vi "Make PUT Object Request Parameters.vi"(11 "PUT Object Request Parameters":T1={"Content Type"="binary/octet-stream", "ACL"=enum."private", "Storage Class"=enum."STANDARD", "User-Defined Metadata"=[]}) -> (3 "HTTP Headers":T4[](array[typedef]))   [LabVIEW 2015, in "NI_AWS_S3.lvlib" / "Object.lvlib"]
uses:
  Object.lvlib
  Core/HTTP Request/Name Value Pair.ctl
  PUT Object Request Parameters.ctl
  ACL.ctl
  Storage Class.ctl
  Core/HTTP Request/HTTP Request.lvclass
  NI_AWS_S3.lvlib
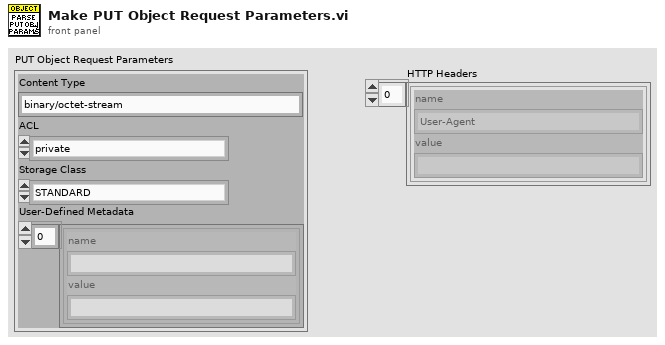
[diagram p1: front panel]
types:
  T1 = typedef "NI_AWS_S3.lvlib/PUT Object Request Parameters.ctl" = cluster{"Content Type":string, "ACL":T2, "Storage Class":T3, "User-Defined Metadata":T4[]}
  T2 = typedef "NI_AWS_S3.lvlib/ACL.ctl" = enum16{"private", "public-read", "public-read-write", "aws-exec-read", "authenticated-read", "bucket-owner-read", "bucket-owner-full-control"}
  T3 = typedef "NI_AWS_S3.lvlib/Storage Class.ctl" = enum16{"STANDARD", "REDUCED_REDUNDANCY"}
  T4 = typedef "NI_AWS_Core.lvlib/HTTP Request.lvclass/Name Value Pair.ctl" = cluster{"name":string, "value":string}
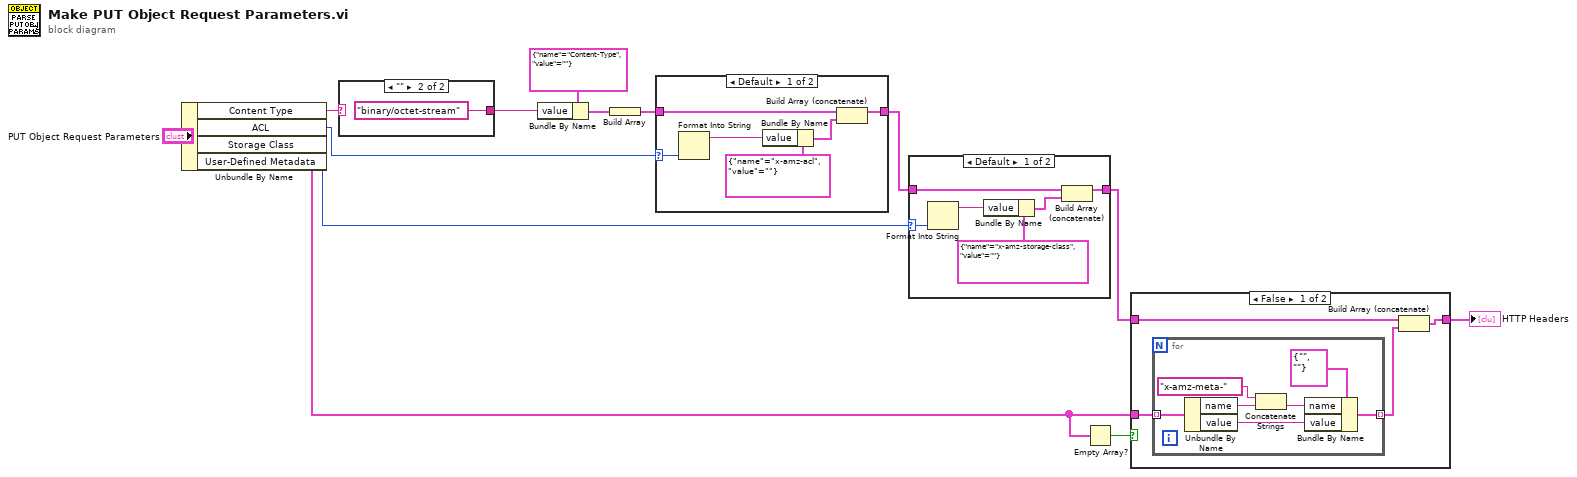
[diagram p0: block diagram]
diagram:
  n1 = Unbundle By Name("PUT Object Request Parameters") -> ("Content Type"=w7:string, "ACL"=w6:T2, "Storage Class"=w5:T3, "User-Defined Metadata"=w1:T4[])
  n2 = case shown="\"\"" w7 {
    selector: w7 -> [w14 _]
    tunnel: [w14 "binary/octet-stream" ("t")] -> w9
    frame Default {
    }
    frame "" {
    }
  }
  n3 = Bundle By Name(cluster=T4 {"name"="Content-Type", "value"=""} ("Name Value Pair"), "value"=w9) -> (w11:T4)
  n4 = Build Array(w11) -> (w8:T4[])
  n5 = case shown="Default" w6 {
    selector: w6 -> [w18 _]
    tunnel: w8 -> [w17 w22]
    tunnel: [w16 w22] -> w4
    frame Default {
      n6 = Format Into String(w18) -> (resulting string=w20:string)  [unwired: 3 in, 1 out]
      n7 = Bundle By Name(cluster=T4 {"name"="x-amz-acl", "value"=""} ("Name Value Pair"), "value"=w20) -> (w21:T4)
      n8 = Build Array (concatenate)(w17, w21) -> (w16:T4[])
    }
    frame "private" {
    }
  }
  n9 = case shown="Default" w5 {
    selector: w5 -> [w26 _]
    tunnel: w4 -> [w25 w29]
    tunnel: [w24 w29] -> w3
    frame Default {
      n10 = Format Into String(w26) -> (resulting string=w28:string)  [unwired: 3 in, 1 out]
      n11 = Bundle By Name(cluster=T4 {"name"="x-amz-storage-class", "value"=""} ("Name Value Pair"), "value"=w28) -> (w23:T4)
      n12 = Build Array (concatenate)(w25, w23) -> (w24:T4[])
    }
    frame "STANDARD" {
    }
  }
  n13 = Empty Array?(array=w1) -> (empty?=w12:bool)
  n14 = case shown="False" w12 {
    tunnel: w1 -> [w33 _]
    tunnel: w3 -> [w32 w41]
    tunnel: [w31 w41] -> w2
    frame False {
      n15 = for {
        tunnel: w33 -> [w40] mode=indexing
        tunnel: [w34] -> w30 mode=indexing
        n16 = Unbundle By Name(w40) -> ("name"=w38:string, "value"=w35:string)
        n17 = Concatenate Strings("x-amz-meta-", w38) -> (w36:string)
        n18 = Bundle By Name(cluster=T4 {"name"="", "value"=""} ("Name Value Pair"), "name"=w36, "value"=w35) -> (w34:T4)
      }
      n19 = Build Array (concatenate)(w32, w30) -> (w31:T4[])
    }
    frame True {
    }
  }
  "HTTP Headers" <- w2
